vi "[ex ce] History of 1D array.vi"() -> ()   [LabVIEW 2021]
doc: "<B>Variable Manager example</B>\n\nThe VI demonstrates a use of variable history for arrays.\n\n::: CalcExpress Toolkit :::\nCopyright (c) 2000-2026 Konstantin Shifershteyn. All rights reserved."
panel:
  out "time 3":dbl format="%<%H:%M:%S%2u\n%d/%m/%Y>T"
  out "graph 3":dbl[](graph)
  in  "reverse order":bool=TRUE
  out "time 2":dbl format="%<%H:%M:%S%2u\n%d/%m/%Y>T"
  out "time 1":dbl format="%<%H:%M:%S%2u\n%d/%m/%Y>T"
  out "time 0":dbl format="%<%H:%M:%S%2u\n%d/%m/%Y>T"
  out "graph 2":dbl[](graph)
  out "graph 1":dbl[](graph)
  out "graph 0":dbl[](graph)
  in  "history length":i32=4
  in  "stop":bool
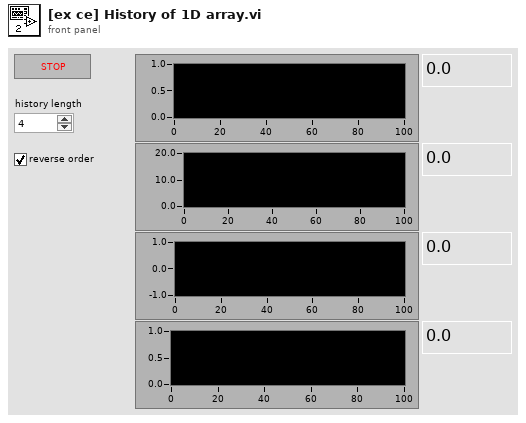
[diagram p1: front panel]
types:
  T1 = enum32{"nop", "create", "destroy", "reset", "get info", "config"}
  T2 = enum16{"create", "destroy", "set value", "get value"}
  T3 = typedef "VarMan Variable Context Handle.ctl" = i32
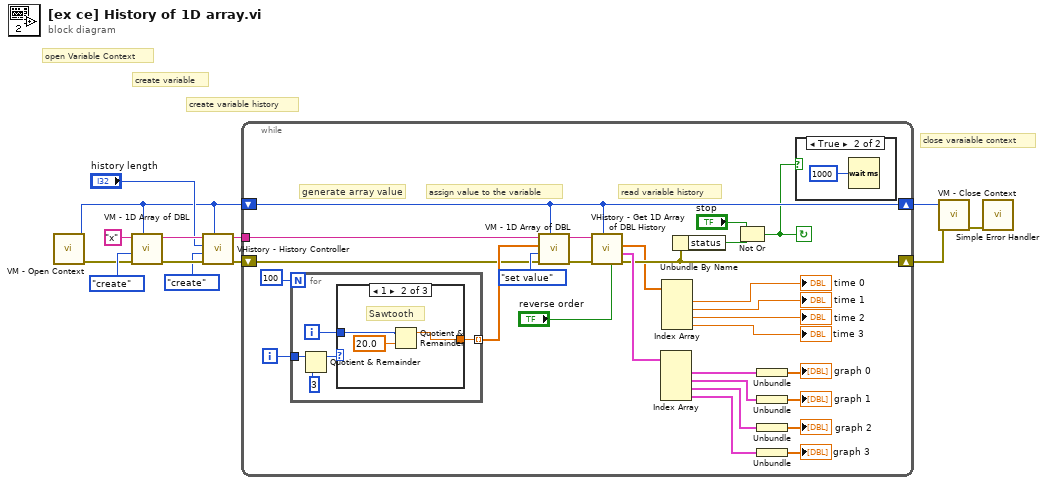
[diagram p0: block diagram]
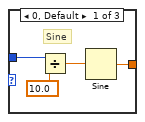
[diagram p3: hidden frame]
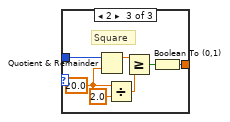
[diagram p4: hidden frame]
diagram:
  # "close varaiable context"
  # "create variable history"
  # "create variable"
  # "open Variable Context"
  n1 = call "VM - Open Context.vi"() -> ("error out"=w10:errorcluster, "VC Handle out"=w5:T3)  [unwired: 9 in, 1 out]
  n2 = call "VM - 1D Array of DBL.vi"("VC Handle"=w5, "error in"=w10, "cmd"=T2."create", "name_spec"="x" ("name")) -> ("error out"=w9:errorcluster, "dup name_spec"=w13:string)  [unwired: 2 in, 4 out]
  n3 = call "VHistory - History Controller.vi"("VC Handle"=w5, "error in"=w9, "cmd (nop:default)"=T1."create", "history length"="history length", "name_spec"=w13) -> ("error out"=w3:errorcluster, "dup name_spec"=w4:string)  [unwired: 3 in, 2 out]
  n4 = while {
    shift-left: w3 -> [w28]
    shift-right: [w27] -> w2
    tunnel: w4 -> [w32]
    shift-left: w5 -> [w33]
    shift-right: [w33] -> w6
    i -> [w30]
    stop <- w14 continue-if-true
    # "read variable history"
    # "assign value to the variable"
    # "generate array value"
    n5 = for {
      N: 100 -> [_]
      tunnel: [w45] -> w29 mode=indexing
      tunnel: w30 -> [w44]
      i -> [w43]
      n6 = Quotient & Remainder(x=w44, y=3) -> (x-y*floor(x/y)=w46:i32)  [unwired: 1 out]
      n7 = case shown="1" w46 {
        tunnel: w43 -> [w51 w54 w61]
        tunnel: [w48 w52 w55] -> w45
        frame 0, Default {
          # "Sine"
          n8 = Divide(x=w51, y=10.0) -> (x/y=w49:dbl)
          n9 = Sine(x=w49) -> (sin(x)=w48:dbl)
        }
        frame 1 {
          # "Sawtooth"
          n10 = Quotient & Remainder(x=w54, y=20.0) -> (x-y*floor(x/y)=w52:dbl)  [unwired: 1 out]
        }
        frame 2 {
          w60 = 20.0 ("y")
          # "Square"
          n11 = Quotient & Remainder(x=w61, y=w60) -> (x-y*floor(x/y)=w58:dbl)  [unwired: 1 out]
          n12 = Divide(x=w60, y=2.0) -> (x/y=w57:dbl)
          n13 = Greater Or Equal?(x=w58, y=w57) -> (x >= y?=w56:bool)
          n14 = Boolean To (0,1)(Boolean=w56) -> (0, 1=w55:i16)
        }
      }
    }
    n15 = call "VM - 1D Array of DBL.vi"("VC Handle"=w33, "error in"=w28, "cmd"=T2."set value", "value in"=w29, "name_spec"=w32) -> ("error out"=w35:errorcluster, "dup name_spec"=w36:string)  [unwired: 1 in, 4 out]
    n16 = call "VHistory - Get 1D Array of DBL History.vi"("reverse order (T)"="reverse order", "VC Handle"=w33, "error in"=w35, "name_spec"=w36) -> ("error out"=w27:errorcluster, "history"=w41:cluster{"data":dbl[]}[], "time stamps"=w21:dbl[])  [unwired: 3 in, 2 out]
    n17 = Index Array(array=w41) -> (element #1=w40:cluster{"data":dbl[]}, element #2=w23:cluster{"data":dbl[]}, element #3=w22:cluster{"data":dbl[]}, element #4=w17:cluster{"data":dbl[]})  [unwired: 4 in]
    n18 = Index Array(array=w21) -> (element #1=→"time 0":dbl, element #2=→"time 1":dbl, element #3=→"time 2":dbl, element #4=→"time 3":dbl)  [unwired: 4 in]
    n19 = Unbundle By Name(w27) -> ("status"=w26:bool)
    n20 = Not Or(1:w26, 2:"stop") -> (0:w14:bool)
    n21 = Unbundle(w40) -> ("data"=→"graph 0":dbl[])
    n22 = Unbundle(w23) -> ("data"=→"graph 1":dbl[])
    n23 = Unbundle(w22) -> ("data"=→"graph 2":dbl[])
    n24 = Unbundle(w17) -> ("data"=→"graph 3":dbl[])
    n25 = case shown="True" w14 {
      frame False {
      }
      frame True {
        n26 = Wait (ms)(milliseconds to wait=u32 1000) -> ()  [unwired: 1 out]
      }
    }
  }
  n27 = call "VM - Close Context.vi"("error in"=w2, "VC Handle"=w6) -> ("error out"=w1:errorcluster)  [unwired: 8 in, 1 out]
  n28 = call <vilib>:"Simple Error Handler.vi"("error in (no error)"=w1) -> ()  [unwired: 4 in, 5 out]
